vi "optical_low_level_get_image_data.vi"() -> ()   [LabVIEW 2025]
uses:
  <vilib>/vision/driver/IMAQdx.llb/IMAQdx Acquisition Mode.ctl
  <vilib>/vision/driver/NI_Vision_Acquisition_Software.lvlib
panel:
  out "Image":T1(plugin-control)
  out "error out":errorcluster
  out "Times between Frames":u32
  in  "Output Folder":path
  in  "Stop":bool
  in  "Camera Name":refnum<k21> caption="IMAQdx Session"
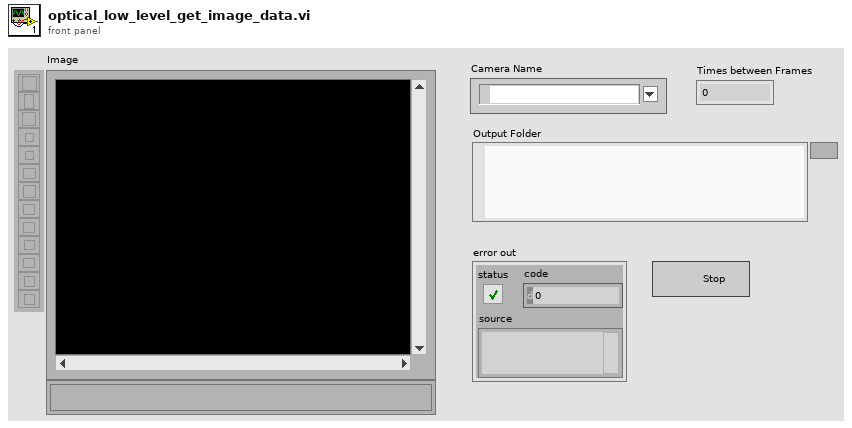
[diagram p1: front panel]
types:
  T1 = typedef "IMAQ Image.ctl" = refnum<image>
  T2 = typedef "Image Type" = u32
  T3 = typedef "NI_Vision_Acquisition_Software.lvlib/IMAQdx Acquisition Mode.ctl" = enum32{"One Shot", "Continuous"}
  T4 = typedef "IMAQdx.ctl" = refnum<k21>
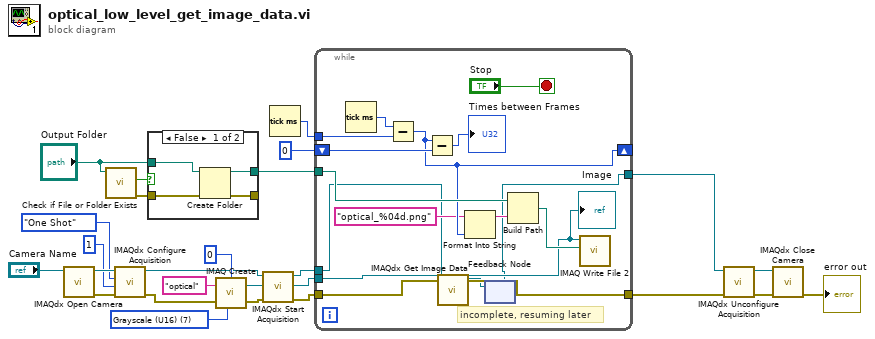
[diagram p0: block diagram]
diagram:
  w10 = T2 7 items=["Grayscale (U8)", "Grayscale (I16)", "Grayscale (SGL)", "Complex (CSG)", "RGB (U32)", "HSL (U32)", "RGB (U64)", "Grayscale (U16)"] ("Image Type")
  n1 = call <vilib>:"IMAQdx Open Camera.vi"("Session In"="Camera Name") -> ("error out"=w18:errorcluster, "Session Out"=w19:T4)  [unwired: 9 in]
  n2 = call <vilib>:"Check if File or Folder Exists.vi"("path"="Output Folder") -> ("error out"=w23:errorcluster, "file or folder exists?"=w25:bool)  [unwired: 8 in, 1 out]
  n3 = call <vilib>:"IMAQdx Configure Acquisition.vi"("error in"=w18, "Number of Buffers"=u32 1, "Continuous?"=IMAQdx_Acquisition_Mode."One Shot", "Session In"=w19) -> ("error out"=w12:errorcluster, "Session Out"=w4:T4)  [unwired: 6 in]
  n4 = case shown="False" w25 {
    tunnel: "Output Folder" -> [w29 w31]
    tunnel: [w28 w31] -> w22
    tunnel: w23 -> [w27 w30]
    tunnel: [w26 w30] -> _
    frame False {
      n5 = Create Folder(path (use dialog)=w29, error in=w27) -> (created path=w28:path, error out=w26:errorcluster)  [unwired: 1 in, 1 out]
    }
    frame True {
    }
  }
  n6 = call "IMAQ Create"("Border Size"=0, "Image Name"="optical", "Image Type"=w10, "error in (no error)"=w12) -> ("New Image"=w13:T1, "error out"=w2:errorcluster)  [unwired: 1 in]
  n7 = call <vilib>:"IMAQdx Start Acquisition.vi"("error in"=w2, "Session In"=w4) -> ("error out"=w1:errorcluster, "Session Out"=w3:T4)  [unwired: 8 in]
  n8 = Tick Count (ms)() -> (millisecond timer value=w21:u32)
  n9 = while {
    tunnel: w22 -> [w46]
    tunnel: w21 -> [w44]
    shift-right: [w41] -> _
    shift-left: u32 0 -> [w42]
    tunnel: w3 -> [w32]
    tunnel: [w33] -> w6
    tunnel: [w37] -> w8
    tunnel: w1 -> [w37]
    tunnel: w13 -> [w36]
    stop <- "Stop" stop-if-true
    # "incomplete, resuming later"
    n10 = Tick Count (ms)() -> (millisecond timer value=w45:u32)
    n11 = Subtract(x=w45, y=w44) -> (x-y=w41:u32)
    n12 = Subtract(x=w41, y=w42) -> (x-y=→"Times between Frames":u32)
    n13 = call <vilib>:"IMAQdx Get Image Data.vi"("Session In"=w32) -> ("Session Out"=w34:T4)  [unwired: 7 in, 3 out]
    n14 = Format Into String(format string="optical_%04d.png", w41) -> (resulting string=w40:string)  [unwired: 2 in, 1 out]
    n15 = feedback-in #1(w34) -> ()
    n16 = feedback #1() -> (w33:T4)  [unwired: 1 in]
    n17 = Build Path(base path=w46, name or relative path=w40) -> (appended path=w38:path)
    n18 = call-poly "IMAQ Write File 2"("File Path"=w38, "Image"=w36) -> ()  [unwired: 8 in, 2 out]
    "Image" <- w36
  }
  n19 = call <vilib>:"IMAQdx Unconfigure Acquisition.vi"("error in"=w8, "Session In"=w6) -> ("error out"=w7:errorcluster, "Session Out"=w5:T4)  [unwired: 8 in]
  n20 = call <vilib>:"IMAQdx Close Camera.vi"("error in"=w7, "Session In"=w5) -> ("error out"=→"error out":errorcluster)  [unwired: 9 in]
